vi "Flush CIF Subscriber.vi"(8 "error in (no error)":errorcluster, 11 "Subscriber Reference":T1 {"refnum" format="%.0x"}) -> (0 "error out":errorcluster, 3 "Discarded":u32)   [LabVIEW 2021, in "Iceoryx.lvlib"]
uses:
  Iceoryx.lvlib
  SubVIs/Convert Error Core.vi
  Refnum/Typedef/CIF Subscriber Refnum.ctl
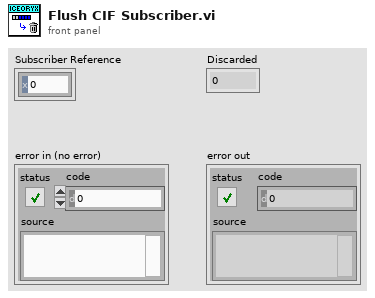
[diagram p1: front panel]
types:
  T1 = typedef "Iceoryx.lvlib/CIF Subscriber Refnum.ctl" = cluster{"refnum":u64, "CIF Sub":enum8{"cifsub"}}
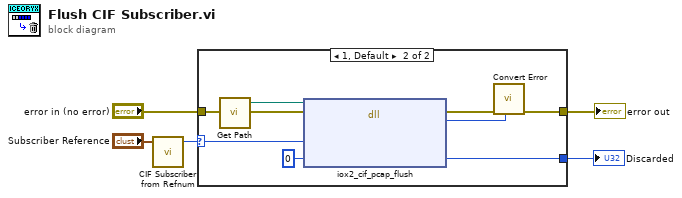
[diagram p0: block diagram]
diagram:
  n1 = call "CIF Subscriber from Refnum.vi"("CIF Subscriber Refnum"="Subscriber Reference") -> ("CIF Subscriber U64"=w1:u64)  [unwired: 4 in]
  n2 = case shown="1, Default" w1 {
    selector: w1 -> [_ w11]
    tunnel: "error in (no error)" -> [w6 w10]
    tunnel: [w6 w9] -> w3
    tunnel: [_ w7] -> w2
    frame 0 {
    }
    frame 1, Default {
      n3 = call "Get Path.vi"() -> ("libiox2_cif path"=w14:path)  [unwired: 4 in]
      n4 = dll-call lib="D:/dev/iceoryx2_lvwrapper/dist/iox2_cif.dll" fn="iox2_cif_pcap_flush"(path in=w14, error in=w10, "subscriber"=w11, "discarded"=u32 0) -> (error out=w13:errorcluster, "return type"=w12:i32, "discarded"=w7:u32)  [unwired: 2 in, 1 out]
      n5 = call "Convert Error.vi"("return type"=w12, "error in (no error)"=w13) -> ("error out"=w9:errorcluster)  [unwired: 9 in]
    }
  }
  "error out" <- w3
  "Discarded" <- w2
